vi "Open File.vi"(8 "error in (no error)":errorcluster caption="错误输入（无错误）", 11 "Data Viewer 输入":refnum<class "Data Viewer.lvclass">) -> (0 "error out":errorcluster caption="错误输出", 3 "Data Viewer 输出":refnum<class "Data Viewer.lvclass">)   [LabVIEW 2020, in "Data Viewer.lvlib" / "Data Viewer.lvclass"]
uses:
  Data Viewer.lvclass
  Data Viewer.lvclass/Data Viewer.ctl
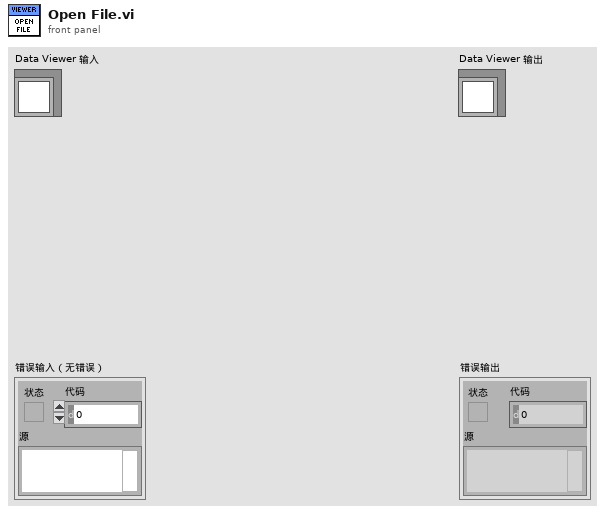
[diagram p1: front panel]
types:
  T1 = typedef "Data Viewer.lvlib/Data Serie--cluster.ctl" = cluster{"Name":string, "Unit":string, "Sample Rate[Hz]":dbl, "Delta t[S]":dbl, "t0":timestamp, "Length":i32, "Time":timestamp[], "Value":dbl[]}
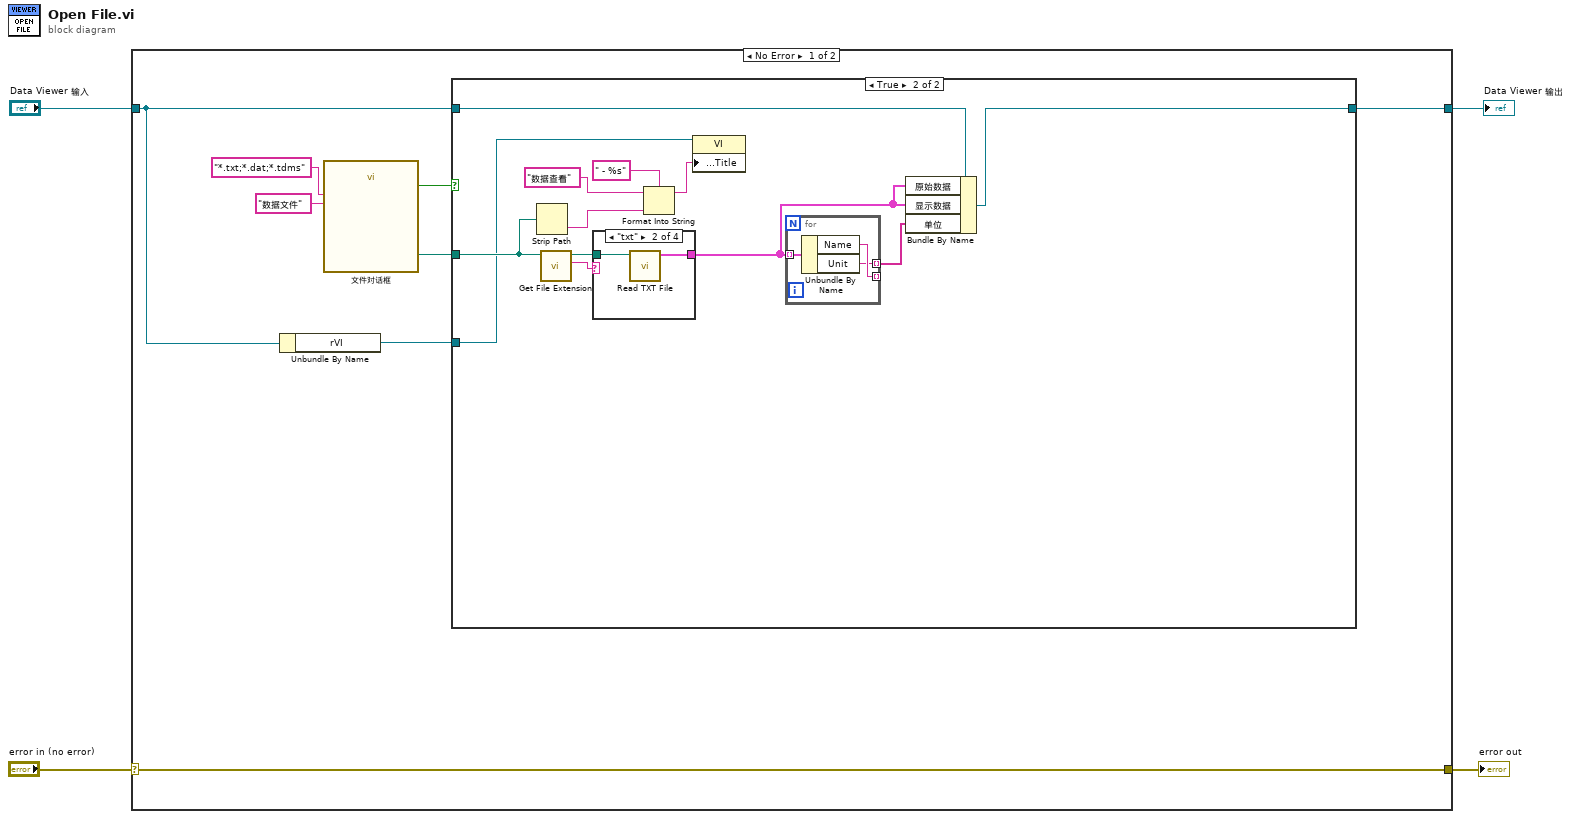
[diagram p0: block diagram]
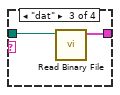
[diagram p4: hidden frame]
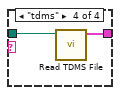
[diagram p5: hidden frame]
diagram:
  n1 = case shown="No Error" "error in (no error)" {
    selector: "error in (no error)" -> [w12 w36]
    tunnel: [w12 w36] -> w3
    tunnel: [w6 w35] -> w1
    tunnel: "Data Viewer 输入" -> [w8 w35]
    frame No Error {
      n2 = Unbundle By Name(w8) -> ("rVI"=w7:refnum<vi>)
      n3 = call "文件对话框"("pattern (all files)"="*.txt;*.dat;*.tdms", "pattern label"="数据文件") -> ("selected path"=w9:path, "exists"=w5:bool)  [unwired: 10 in, 2 out]
      n4 = case shown="True" w5 {
        tunnel: w9 -> [_ w25]
        tunnel: w8 -> [w13 w24]
        tunnel: w7 -> [_ w23]
        tunnel: [w13 w22] -> w6
        frame False {
        }
        frame True {
          n5 = Strip Path(path=w25) -> (name=w16:string)  [unwired: 1 out]
          n6 = call <vilib>:"Get File Extension.vi"("file"=w25) -> ("lowercase file extension"=w18:string, "dup file"=w17:path)  [unwired: 6 in, 3 out]
          n7 = case shown="\"txt\"" w18 {
            tunnel: w17 -> [_ w27 w29 w31]
            tunnel: [_ w26 w28 w30] -> w20
            frame "假", Default {
            }
            frame "txt" {
              n8 = call "Read TXT File.vi"("File Path"=w27) -> ("数据系列"=w26:T1[])  [unwired: 10 in]
            }
            frame "dat" {
              n9 = call "Read Binary File.vi"("路径"=w29) -> ("数据系列"=w28:T1[])  [unwired: 9 in, 1 out]
            }
            frame "tdms" {
              n10 = call "Read TDMS File.vi"("文件路径"=w31) -> ("数据系列"=w30:T1[])  [unwired: 10 in]
            }
          }
          n11 = Format Into String(format string=" - %s" ("格式字符串"), initial string="数据查看" ("初始字符串"), w16) -> (resulting string=w19:string)  [unwired: 1 in, 1 out]
          n12 = property class="VI"(reference=w23, "Front Panel.Title"=w19) -> ()  [unwired: 1 in, 2 out]
          n13 = for {
            tunnel: w20 -> [w34] mode=indexing
            tunnel: [w33] -> _ mode=indexing
            tunnel: [w32] -> w21 mode=indexing
            n14 = Unbundle By Name(w34) -> ("Name"=w33:string, "Unit"=w32:string)
          }
          n15 = Bundle By Name(cluster=w24, "原始数据"=w20, "显示数据"=w20, "单位"=w21) -> (w22:refnum<class "Data Viewer.lvclass">)
        }
      }
    }
    frame Error {
    }
  }
  "error out" <- w3
  "Data Viewer 输出" <- w1
